vi "FuncVI_Sub - Probe - Set window position.vi"(7 "Master VI Ref":refnum<vi>, 8 "error in":errorcluster, 10 "left-top corner":cluster{"x":i16, "y":i16}={"x"=-1, "y"=-1}, 11 "VI RefNum":refnum<vi>) -> (0 "error out":errorcluster, 3 "dup VI Refnum":refnum<vi>)   [LabVIEW 2021]
doc: "::: CalcExpress Toolkit :::\nCopyright (c) 2000-2026 Konstantin Shifershteyn. All rights reserved."
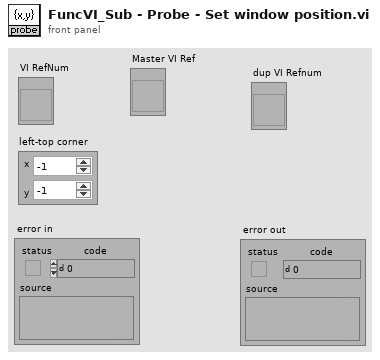
[diagram p1: front panel]
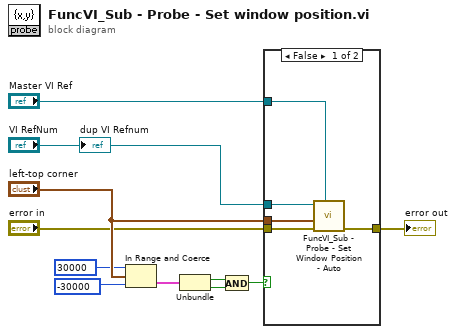
[diagram p0: block diagram]
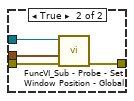
[diagram p2: hidden frame]
diagram:
  n1 = In Range and Coerce(upper limit=i16 30000 ("x"), x="left-top corner", lower limit=i16 -30000 ("x")) -> (In Range?=w3:cluster{"x":bool, "y":bool})  [unwired: 1 out]
  n2 = Unbundle(w3) -> ("x"=w4:bool, "y"=w5:bool)
  n3 = And(x=w4, y=w5) -> (x .and. y?=w6:bool)
  n4 = case shown="False" w6 {
    tunnel: "VI RefNum" -> [w14 w20]
    tunnel: "error in" -> [w16 w19]
    tunnel: [w15 w18] -> w11
    tunnel: "left-top corner" -> [w13 w17]
    tunnel: "Master VI Ref" -> [w12 _]
    frame False {
      n5 = call "FuncVI_Sub - Probe - Set Window Position - Auto .vi"("Master VI Ref"=w12, "error in"=w16, "Window Position"=w13, "Probe VI Ref"=w14) -> ("error out"=w15:errorcluster)  [unwired: 6 in, 1 out]
    }
    frame True {
      n6 = call "FuncVI_Sub - Probe - Set Window Position - Global.vi"("error in"=w19, "Window Position"=w17, "VI Refnum"=w20) -> ("error out"=w18:errorcluster)  [unwired: 7 in, 1 out]
    }
  }
  "error out" <- w11
  "dup VI Refnum" <- "VI RefNum"
